vi "RDC-error_check.vi"(10 "Reference":cdb[](array[numeric]), 11 "Calculated":cdb[](array[numeric])) -> (3 "Error Metric":T1)   [LabVIEW 2020, in "RDC-Reflection_Data_Computation.lvlib"]
doc: "Compares a calculated complex array with a reference array and returns an error metric cluster: difference, percent difference, average difference, percent average difference and RMSE difference."
uses:
  RDC-Reflection_Data_Computation.lvlib
  RDC-error_metric_clust.ctl
  4fbbaee8-9426-4521-b562-7bee34f26c6b.vi
  00b2f8b2-42fb-4ba9-ad79-5185982ba082.vi
  cdf4440f-7c1a-473f-9453-edadec0e90b2.vi
  3eee7f0e-e172-47cd-aa51-018769cf2cc4.vi
  9aaa4270-96ba-4dce-ad12-645d88e50467.vi
  93ba1d51-08c2-452e-83ad-b1e7530e918d.vi
panel:
  out "percent diff":cdb[](array[numeric])
  out "Percent avg diff":cdb
  out "RMSE diff":cdb
  out "Diff":cdb[](array[numeric])
  out "Average diff":cdb
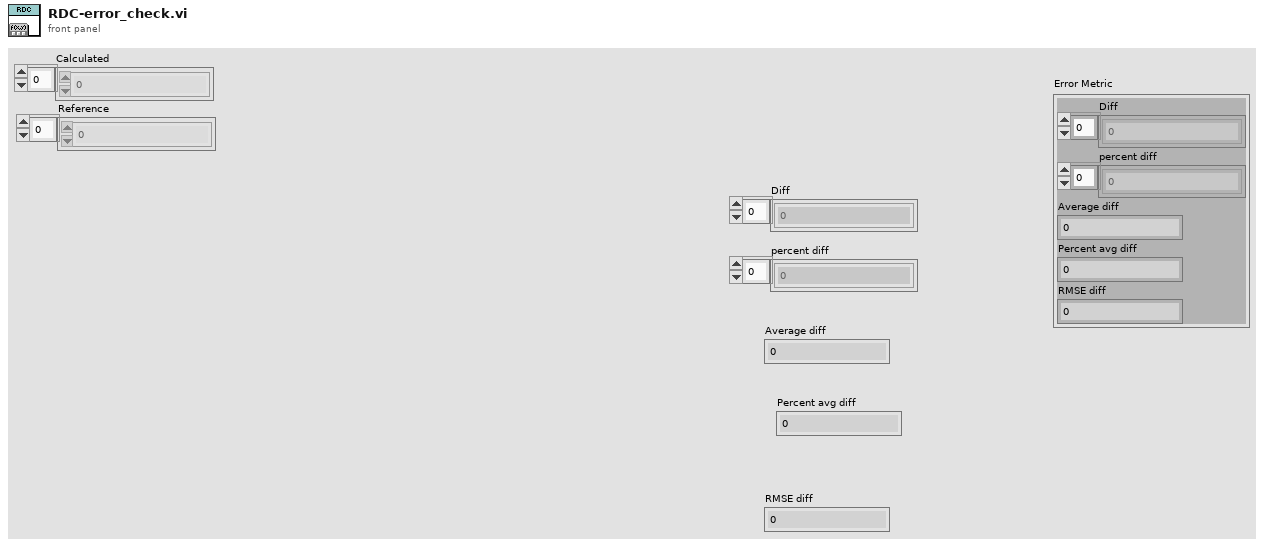
[diagram p1: front panel]
types:
  T1 = typedef "RDC-Reflection_Data_Computation.lvlib/RDC-error_metric_clust.ctl" = cluster{"Diff":cdb[], "percent diff":cdb[], "Average diff":cdb, "Percent avg diff":cdb, "RMSE diff":cdb}
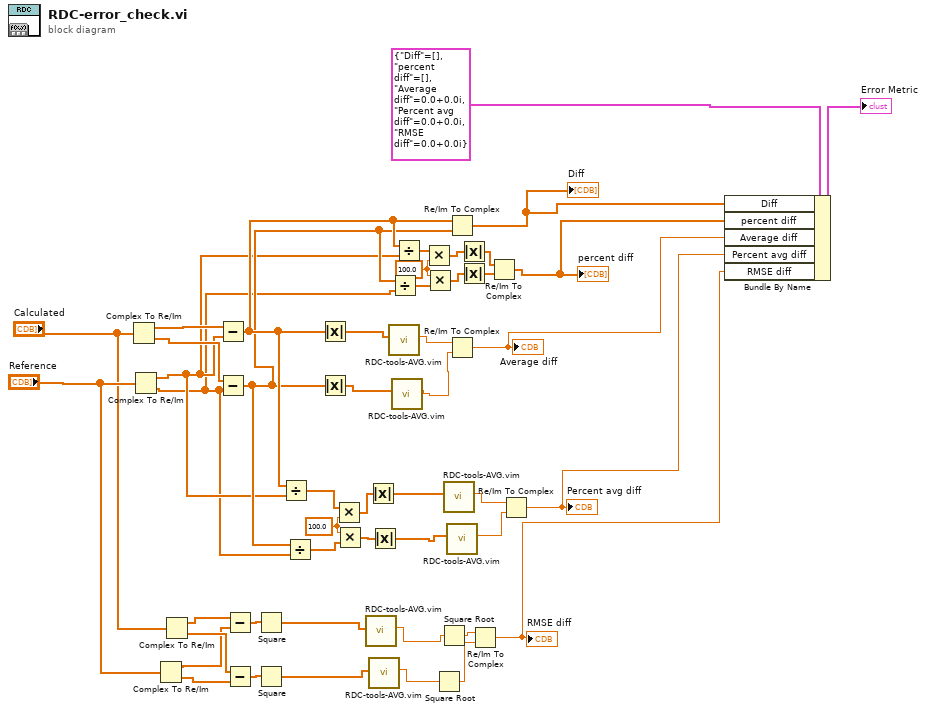
[diagram p0: block diagram]
diagram:
  w38 = 100.0 ("x/y")
  w39 = 100.0 ("x/y")
  n1 = Complex To Re/Im(x + iy="Calculated") -> (x=w33:dbl[], y=w32:dbl[])
  n2 = Complex To Re/Im(x + iy="Reference") -> (x=w31:dbl[], y=w30:dbl[])
  n3 = Complex To Re/Im(x + iy="Reference") -> (x=w25:dbl[], y=w24:dbl[])
  n4 = Complex To Re/Im(x + iy="Calculated") -> (x=w27:dbl[], y=w26:dbl[])
  n5 = Subtract(x=w33, y=w31) -> (x-y=w43:dbl[])
  n6 = Subtract(x=w32, y=w30) -> (x-y=w42:dbl[])
  n7 = Subtract(x=w27, y=w25) -> (x-y=w46:dbl[])
  n8 = Subtract(x=w26, y=w24) -> (x-y=w47:dbl[])
  n9 = Square(x=w46) -> (x^2=w9:dbl[])
  n10 = Square(x=w47) -> (x^2=w6:dbl[])
  n11 = Divide(x=w43, y=w31) -> (x/y=w37:dbl[])
  n12 = Divide(x=w42, y=w30) -> (x/y=w36:dbl[])
  n13 = Absolute Value(x=w43) -> (abs(x)=w17:dbl[])
  n14 = Absolute Value(x=w42) -> (abs(x)=w15:dbl[])
  n15 = Multiply(x=w37, y=w38) -> (x*y=w34:dbl[])
  n16 = Multiply(x=w38, y=w36) -> (x*y=w35:dbl[])
  n17 = call "RDC-tools-AVG.vim"("Data Array"=w9) -> ("AVG"=w8:dbl)  [unwired: 10 in]
  n18 = Absolute Value(x=w34) -> (abs(x)=w13:dbl[])
  n19 = call "RDC-tools-AVG.vim"("Data Array"=w6) -> ("AVG"=w7:dbl)  [unwired: 10 in]
  n20 = Absolute Value(x=w35) -> (abs(x)=w11:dbl[])
  n21 = call "RDC-tools-AVG.vim"("Data Array"=w17) -> ("AVG"=w16:dbl)  [unwired: 10 in]
  n22 = Divide(x=w42, y=w30) -> (x/y=w40:dbl[])
  n23 = call "RDC-tools-AVG.vim"("Data Array"=w15) -> ("AVG"=w14:dbl)  [unwired: 10 in]
  n24 = Divide(x=w43, y=w31) -> (x/y=w41:dbl[])
  n25 = Multiply(x=w41, y=w39) -> (x*y=w5:dbl[])
  n26 = Multiply(x=w39, y=w40) -> (x*y=w2:dbl[])
  n27 = Square Root(x=w7) -> (sqrt(x)=w44:dbl)
  n28 = Square Root(x=w8) -> (sqrt(x)=w45:dbl)
  n29 = call "RDC-tools-AVG.vim"("Data Array"=w13) -> ("AVG"=w12:dbl)  [unwired: 10 in]
  n30 = Re/Im To Complex(1:w42, 2:w43) -> (0:w21:cdb[])
  "Diff" <- w21
  n31 = Re/Im To Complex(1:w14, 2:w16) -> (0:w20:cdb)
  "Average diff" <- w20
  n32 = call "RDC-tools-AVG.vim"("Data Array"=w11) -> ("AVG"=w10:dbl)  [unwired: 10 in]
  n33 = Absolute Value(x=w5) -> (abs(x)=w4:dbl[])
  n34 = Absolute Value(x=w2) -> (abs(x)=w3:dbl[])
  n35 = Re/Im To Complex(1:w44, 2:w45) -> (0:w18:cdb)
  "RMSE diff" <- w18
  n36 = Re/Im To Complex(1:w3, 2:w4) -> (0:w1:cdb[])
  "percent diff" <- w1
  n37 = Re/Im To Complex(1:w10, 2:w12) -> (0:w19:cdb)
  "Percent avg diff" <- w19
  n38 = Bundle By Name(cluster=T1 {"Diff"=[], "percent diff"=[], "Average diff"=0.0+0.0i, "Percent avg diff"=0.0+0.0i, "RMSE diff"=0.0+0.0i} ("Error Metric"), "Diff"=w21, "percent diff"=w1, "Average diff"=w20, "Percent avg diff"=w19, "RMSE diff"=w18) -> (→"Error Metric":T1)
